vi "RichToFlatcif_can_writer_cansub_CansubDevices.vi"(5 "OutputClusterType":T1, 11 "InputCluster":T3) -> (3 "OutputCluster":T1)   [LabVIEW 2021, in "CanWriterCansub_server.lvlib"]
uses:
  CanWriterCansub_server.lvlib
  cif_can_writer_cansub_CansubDevices.ctl
  cif_can_writer_cansub_CansubDevice.ctl
  cif_can_writer_cansub_CansubDevices_Flat.ctl
  cif_can_writer_cansub_CansubDevice_Flat.ctl
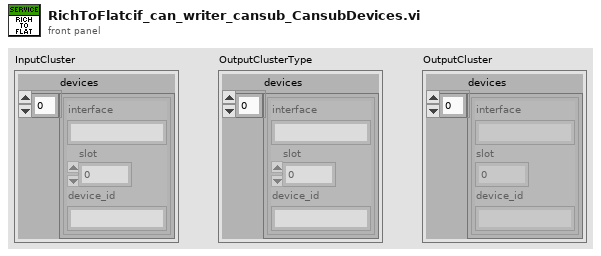
[diagram p1: front panel]
types:
  T1 = typedef "CanWriterCansub_server.lvlib/cif_can_writer_cansub_CansubDevices_Flat.ctl" = cluster{"devices":T2[]}
  T2 = typedef "CanWriterCansub_server.lvlib/cif_can_writer_cansub_CansubDevice_Flat.ctl" = cluster{"interface":string, "slot":u32, "device_id":string}
  T3 = typedef "CanWriterCansub_server.lvlib/cif_can_writer_cansub_CansubDevices.ctl" = cluster{"devices":T4[]}
  T4 = typedef "CanWriterCansub_server.lvlib/cif_can_writer_cansub_CansubDevice.ctl" = cluster{"interface":string, "slot":u32, "device_id":string}
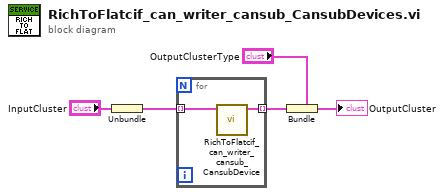
[diagram p0: block diagram]
diagram:
  n1 = Unbundle "Unbundle"("InputCluster") -> ("devices"=w2:T4[])
  n2 = for {
    tunnel: w2 -> [w7] mode=indexing
    tunnel: [w6] -> w1 mode=indexing
    n3 = call "RichToFlatcif_can_writer_cansub_CansubDevice.vi"("InputCluster"=w7) -> ("OutputCluster"=w6:T2)  [unwired: 10 in]
  }
  n4 = Bundle "Bundle"(cluster="OutputClusterType", "devices"=w1) -> (→"OutputCluster":T1)
